vi "RDV-GUI-Compare_Permittivity_calc.vi"() -> ()   [LabVIEW 2020]
doc: "Main viewer, run by hand: loads measurement folders and reference files and compares reflection, impedance and permittivity of every calculation method on graphs and Smith plots, with error analysis. The user picks the folders, the files to compare and the plots to show."
uses:
  RDV-INFO_DATA.ctl
  RDV-UPDATE_IGNORE_LIST.ctl
  Computation/RDC-perm_calc_type.ctl
  RDV-Reflection_Data_viewer.lvclass
  RDV-PRELAUNCH_DATA.ctl
  RDV-XY_GRAPH_REFS.ctl
  RDV-GUI_REFS.ctl
  RDV-PLOT_SETTINGS.ctl
  dedf462c-48f1-4407-ad15-524a3be17598.vi
  Computation/RDC-Reflection_Data_Computation.lvlib
panel:
  out "Selector":T1(graph)
  in  "filter":bool
  in  "unfilter":bool
  in  "Lower Cut-Off":dbl=30000.0 format="%#_13g"
  in  "Calc % error":bool
  in  "Autoscale":bool
  in  "Toggle Plot":bool
  in  "Stop":bool
  in  "Tab Control":T2(tab)
  out "Reflection imag":T1(graph)
  out "Reflection Real":T1(graph)
  out "Impedance imag":T1(graph)
  out "Impedance Real":T1(graph)
  out "Impedance":picture
  out "Permittivity imag":T1(graph)
  out "Permittivity Real":T1(graph)
  out "real error tot":dbl[](array[numeric])
  in  "Reference":u16(ring)=2 items=["00-open0-r", "01-short1-r", "02-water2-r", "03-adblue3-r", "04-eth-124-r", "05-eth-245-r", "06-saline6-r", "07-eth-337-r", "08-eth-488-r", "09-eth-669-r", "10-eth-9610-r", "11-gaba-0111-r", "12-gaba-0512-r", "13-gaba-113-r", "14-iso-1214-r", "15-iso-2515-r", "16-iso-5016-r", "17-iso-9917-r", "18-saline-0p918-r", "19-saline-1-319-r"]
  out "Analyse real":cluster{"Frequency":dbl[], "Perm":dbl[]}[](graph)
  out "Analyse imag":cluster{"Frequency":dbl[], "Perm 2":dbl[]}[](graph)
  out "imag Error":dbl[](array[numeric]) format="%#_6p"
  out "real error":dbl[](array[numeric]) format="%#_6p"
  out "imag error tot":dbl[](array[numeric])
  in  "Data Sets":u16(ring)=1 items=["0-P1_eth-12", "1-P1_eth-24", "2-P1_eth-33", "3-P1_eth-48-2", "4-P1_eth-66", "5-P1_eth-96"]
  in  "Compare Array 2":cluster{"ref":i32, "Set":i32}[](array[cluster])=[{"ref"=0, "Set"=0}, {"ref"=3, "Set"=1}, {"ref"=3, "Set"=2}]
  out "Calculation type":T3[](array[typedef])
  in  "Association set":cluster{"ref":i32, "Set":i32}[](array[cluster])=[{"ref"=3, "Set"=0}, {"ref"=4, "Set"=8}, {"ref"=5, "Set"=10}, {"ref"=7, "Set"=7}, {"ref"=8, "Set"=4}, {"ref"=9, "Set"=3}, {"ref"=10, "Set"=2}, {"ref"=11, "Set"=5}, {"ref"=12, "Set"=6}, {"ref"=13, "Set"=1}, {"ref"=14, "Set"=9}]
  out "compare":T4
  out "Sets of data":string[](array[string])
  out "Total Error real":dbl[](array[numeric])
  out "Total Error Imag":dbl[](array[numeric])
  out "Total Error":dbl[](array[numeric])
  out "All Error imag":dbl[][](array[numeric])
  out "All Error real":dbl[][](array[numeric])
  out "Measurement Param":T5[](array[typedef]) {"lenght" format="%#_6p"; "cap" format="%#_6p"; "Tau" format="%#_6p"}
  in  "Refresh data":bool
  in  "reference paths - Ideal data":path
  in  "common name to remove":string
  in  "max Size":i32=25
  in  "Files for analyses - Data to compare":path
  out "error out":errorcluster
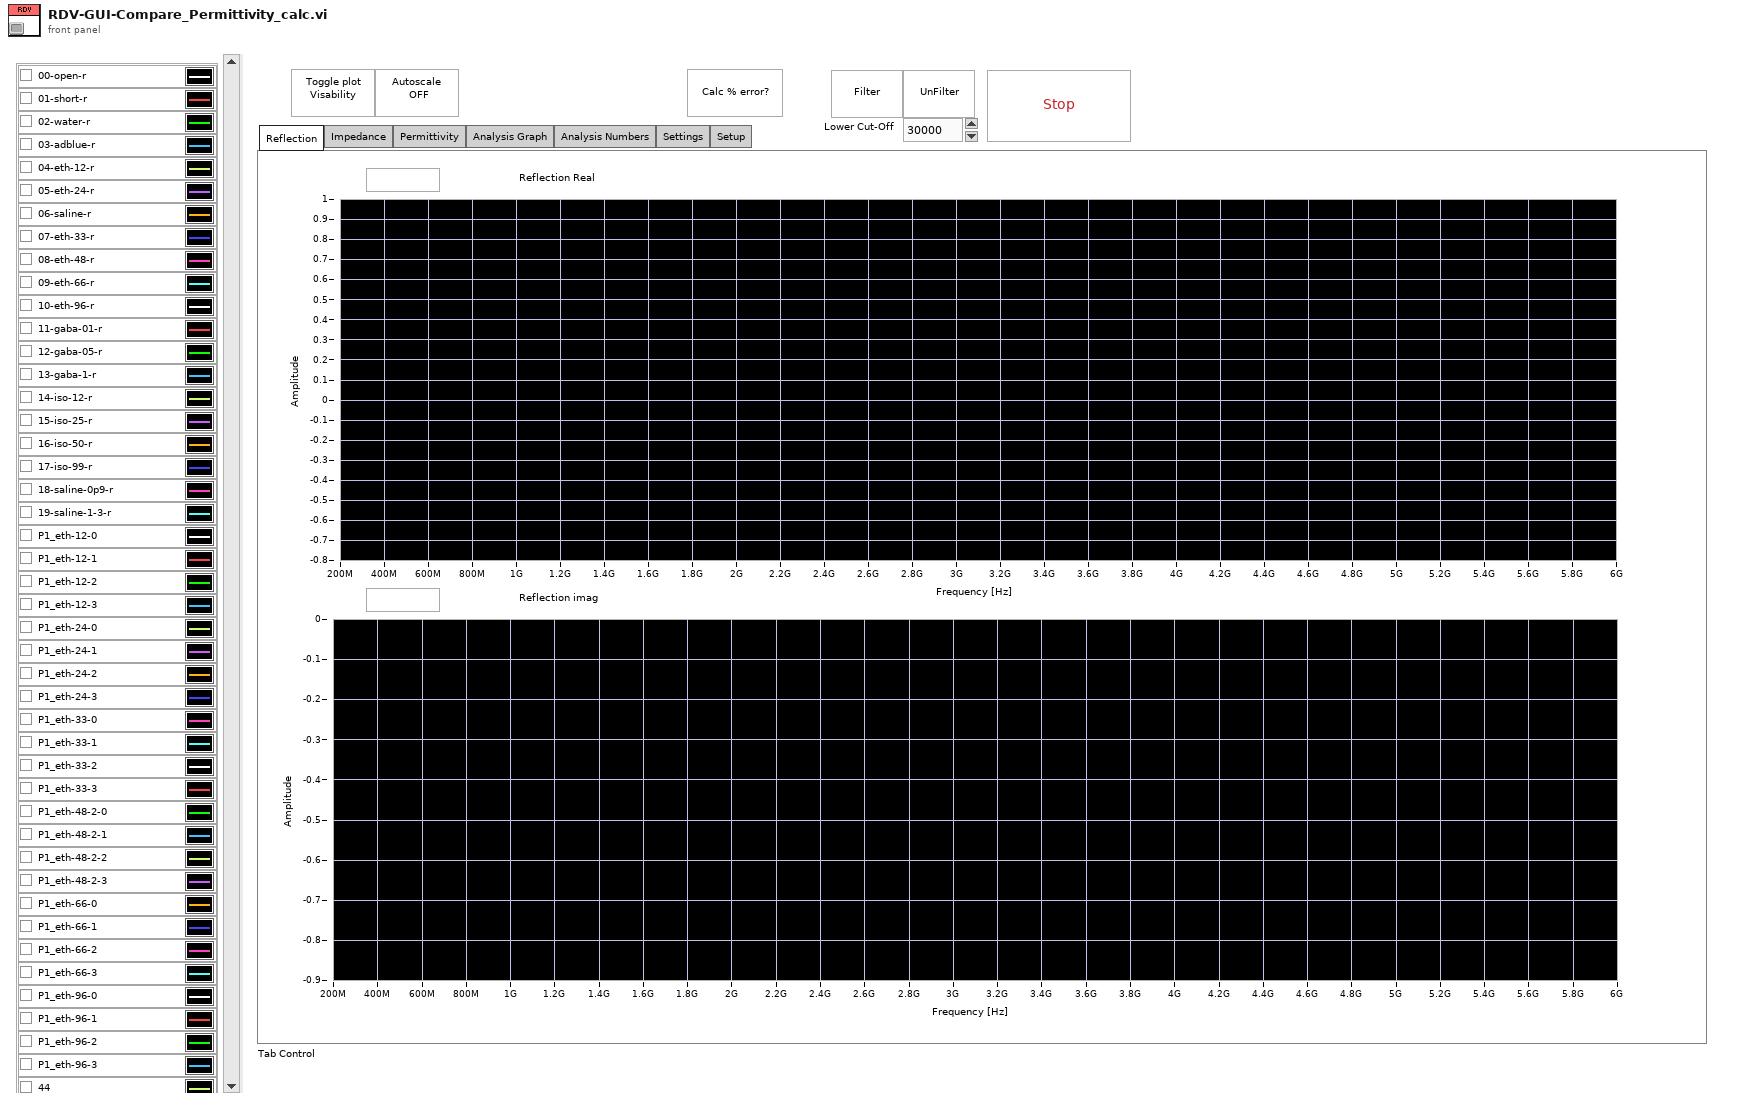
[diagram p1: front panel]
types:
  T1 = cluster{"Frequency":dbl[], "Reflection'":dbl[]}[]
  T2 = enum32{"Reflection", "Impedance", "Permittivity", "Analysis Graph", "Analysis Numbers", "Settings", "Setup"}
  T3 = typedef "RDC-Reflection_Data_Computation.lvlib/RDC-perm_calc_type.ctl" = enum16{"Basic", "Capacative", "Advance", "Bilinear", "Size"}
  T4 = typedef "RDV-Reflection_Data_viewer.lvclass/RDV-UPDATE_IGNORE_LIST.ctl" = string[]
  T5 = typedef "RDV-Reflection_Data_viewer.lvclass/RDV-INFO_DATA.ctl" = cluster{"Name":string, "Tau":dbl, "cap":dbl, "lenght":dbl}
  T6 = typedef "RDV-Reflection_Data_viewer.lvclass/RDV-PLOT_SETTINGS.ctl" = cluster{"common name to remove":string, "Max Size":i32}
  T7 = typedef "RDV-Reflection_Data_viewer.lvclass/RDV-PRELAUNCH_DATA.ctl" = cluster{"XY graph refs":T8, "GUI Refs":T9}
  T8 = typedef "RDV-Reflection_Data_viewer.lvclass/RDV-XY_GRAPH_REFS.ctl" = cluster{"Reflection Real":refnum<vi>, "Reflection Imag":refnum<vi>, "Permittivity Real":refnum<vi>, "Permittivity Imag":refnum<vi>, "Impedance Real":refnum<vi>, "Impedance Imag":refnum<vi>}
  T9 = typedef "RDV-Reflection_Data_viewer.lvclass/RDV-GUI_REFS.ctl" = cluster{"Autoscale":refnum<vi>, "sgl plot Selector":refnum<vi>[], "Smith Plot":refnum<vi>, "plot vis master ":refnum<vi>}
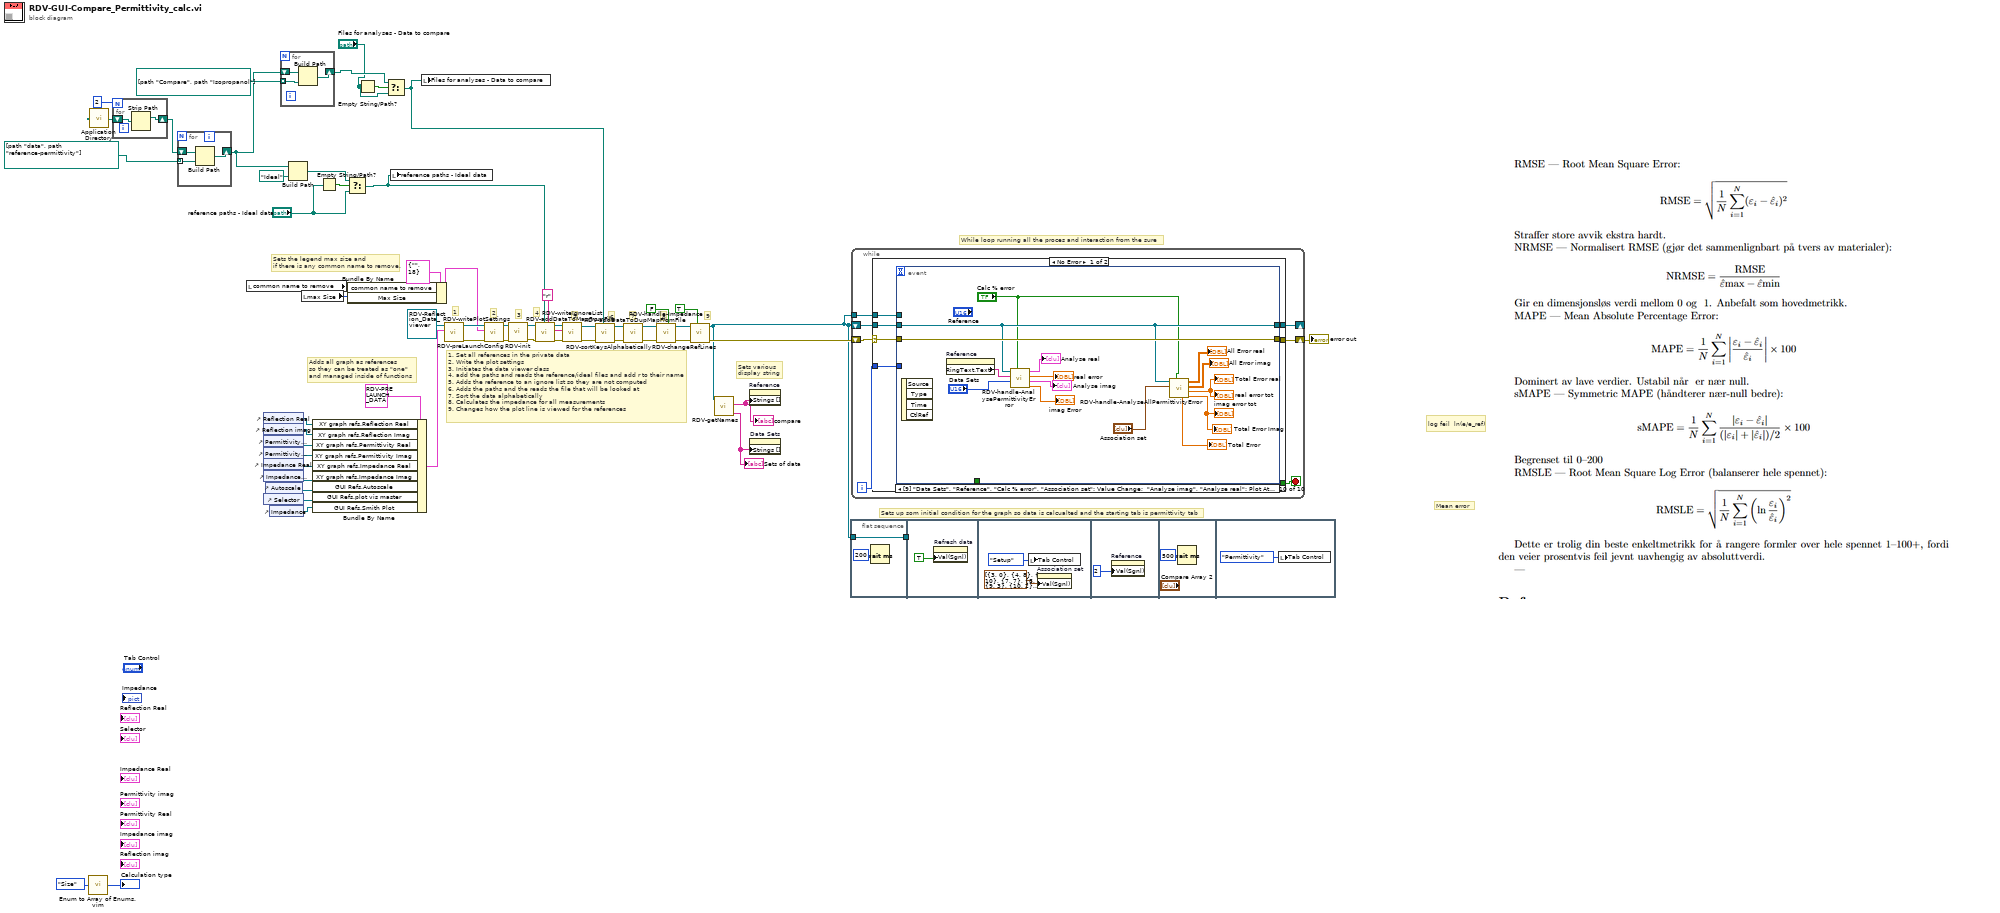
[diagram p0: block diagram]
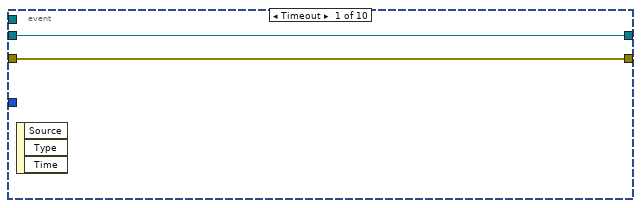
[diagram p2: hidden frame]
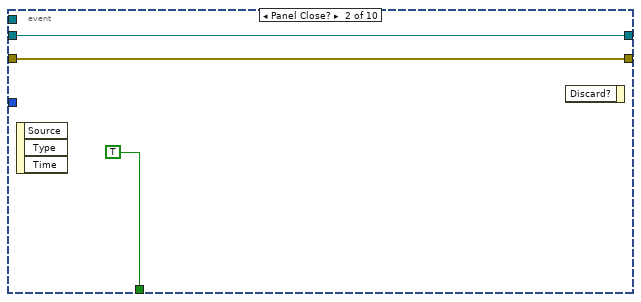
[diagram p3: hidden frame]
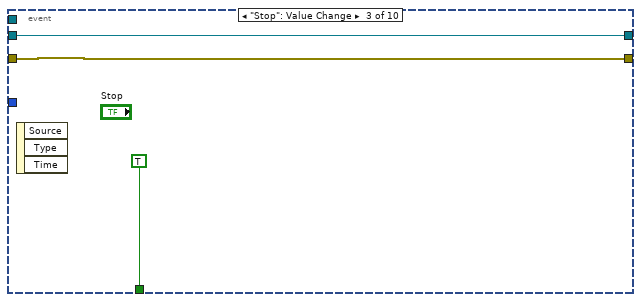
[diagram p4: hidden frame]
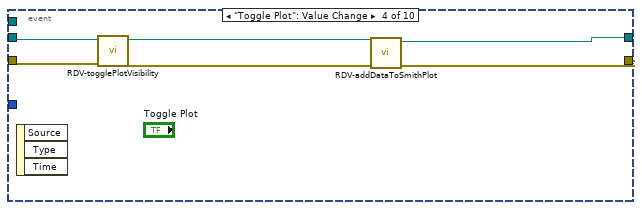
[diagram p5: hidden frame]
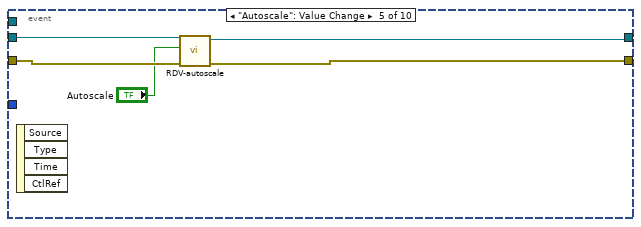
[diagram p6: hidden frame]
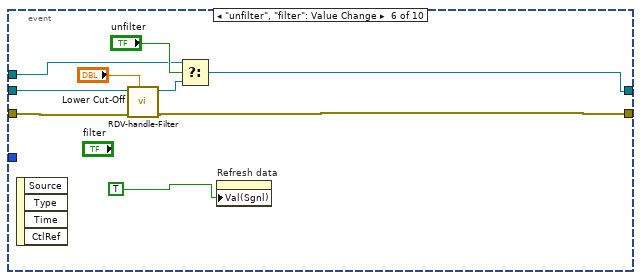
[diagram p7: hidden frame]
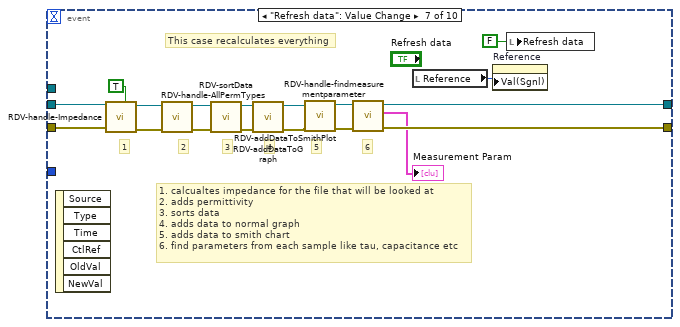
[diagram p8: hidden frame]
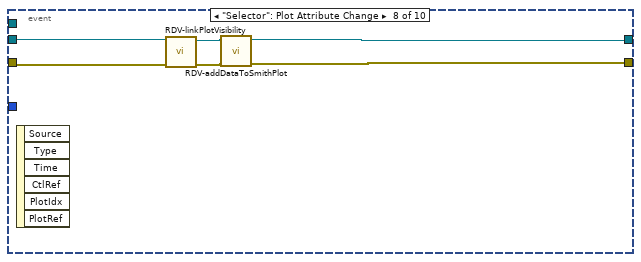
[diagram p9: hidden frame]
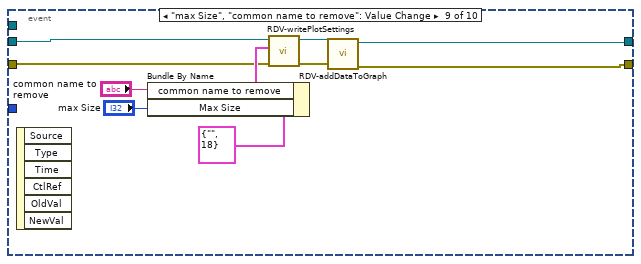
[diagram p10: hidden frame]
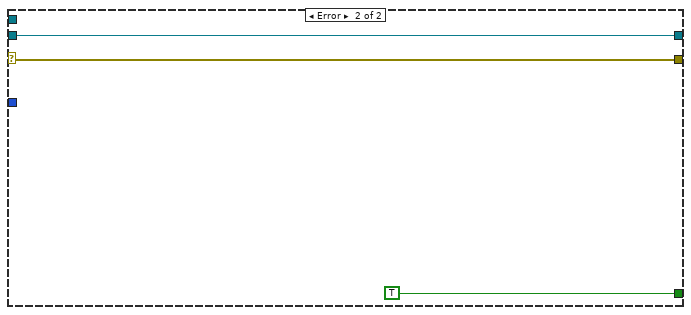
[diagram p11: hidden frame]
diagram:
  # "1. Set all references in the private data\n2. Write the plot settings\n3. Initiates the data viewer class\n4. add the paths and reads the reference/ideal files and add r to their name\n5. Adds the reference to an ignore list so they are not computed\n6. Adds the paths and the reads the file that will be looked at\n7. Sort the data alphabetically\n8. Calculates the impedance for all measurements\n9. Changes how the plot line is viewed for the references"
  # "9"
  # "8"
  # "7"
  # "6"
  # "5"
  # "4"
  # "3"
  # "2"
  # "1"
  # "Sets the legend max size and\nif there is any common name to remove."
  # "Adds all graph as references\nso they can be treated as \"one\"\nand managed inside of functions"
  # "Sets various\ndisplay string"
  # "While loop running all the proces and interaction from the sure"
  # "Sets up som initial condition for the graph so data is calcualted and the starting tab is permittivity tab"
  # "Mean error"
  # "log feil  ln(e/e_ref)"
  n1 = call "Enum to Array of Enums.vim"("enum"=RDC-perm_calc_type."Size" ("Perm calc type")) -> ("array of enums"=→"Calculation type":T3[])
  n2 = call <vilib>:"Application Directory.vi"() -> ("Application Directory"=w13:path)
  n3 = for {
    N: 2 -> [_]
    shift-right: [w60] -> w12
    shift-left: w13 -> [w61]
    n4 = Strip Path(path=w61) -> (stripped path=w60:path)  [unwired: 1 out]
  }
  n5 = for {
    shift-right: [w63] -> w8
    shift-left: w12 -> [w64]
    tunnel: path[] [path "data", path "reference-permittivity"] ("Application Directory") -> [w62] mode=indexing
    n6 = Build Path(base path=w64, name or relative path=w62) -> (appended path=w63:path)
  }
  n7 = local read "common name to remove"() -> (w38:string)
  n8 = control-ref of="Reflection Real"() -> (w52:refnum<vi>)
  n9 = control-ref of="Reflection imag"() -> (w49:refnum<vi>)
  n10 = control-ref of="Permittivity Real"() -> (w48:refnum<vi>)
  n11 = control-ref of="Permittivity imag"() -> (w47:refnum<vi>)
  n12 = control-ref of="Impedance Real"() -> (w46:refnum<vi>)
  n13 = control-ref of="Impedance imag"() -> (w45:refnum<vi>)
  n14 = control-ref of="Selector"() -> (w53:refnum<vi>)
  n15 = control-ref of="Autoscale"() -> (w54:refnum<vi>)
  n16 = control-ref of="Impedance"() -> (w55:refnum<vi>)
  n17 = for {
    shift-right: [w66] -> w4
    shift-left: w8 -> [w67]
    tunnel: path[] [path "Compare", path "Isopropanol"] ("Application Directory") -> [w65] mode=indexing
    n18 = Build Path(base path=w67, name or relative path=w65) -> (appended path=w66:path)
  }
  n19 = Build Path(base path=w8, name or relative path=path "Ideal") -> (appended path=w6:path)
  n20 = local read "max Size"() -> (w37:i32)
  n21 = Bundle By Name(cluster=T7 {"XY graph refs"={"Reflection Real"=refnum, "Reflection Imag"=refnum, "Permittivity Real"=refnum, "Permittivity Imag"=refnum, "Impedance Real"=refnum, "Impedance Imag"=refnum}, "GUI Refs"={"Autoscale"=refnum, "sgl plot Selector"=[], "Smith Plot"=refnum, "plot vis master "=refnum}} ("preLaunch Config"), "XY graph refs.Reflection Real"=w52, "XY graph refs.Reflection Imag"=w49, "XY graph refs.Permittivity Real"=w48, "XY graph refs.Permittivity Imag"=w47, "XY graph refs.Impedance Real"=w46, "XY graph refs.Impedance Imag"=w45, "GUI Refs.Autoscale"=w54, "GUI Refs.plot vis master"=w53, "GUI Refs.Smith Plot"=w55) -> (w56:T7)
  n22 = Empty String/Path?(string/path="reference paths - Ideal data") -> (empty?=w15:bool)
  n23 = Bundle By Name(cluster=T6 {"common name to remove"="", "Max Size"=18} ("Plot Settings"), "common name to remove"=w38, "Max Size"=w37) -> (w39:T6)
  n24 = Select(t=w6, s=w15, f="reference paths - Ideal data") -> (s? t:f=w1:path)
  n25 = Empty String/Path?(string/path="Files for analyses - Data to compare") -> (empty?=w5:bool)
  n26 = Select(t=w4, s=w5, f="Files for analyses - Data to compare") -> (s? t:f=w2:path)
  n27 = local write "reference paths - Ideal data"(w1) -> ()
  n28 = local write "Files for analyses - Data to compare"(w2) -> ()
  n29 = call "RDV-preLaunchConfig.vi"("preLaunch Config"=w56, "RDV-Reflection_Data_viewer in"=refnum<class "RDV-Reflection_Data_viewer.lvclass"> refnum) -> ("error out"=w43:errorcluster, "RDV-Reflection_Data_viewer out"=w44:refnum<class "RDV-Reflection_Data_viewer.lvclass">)  [unwired: 8 in]
  n30 = call "RDV-writePlotSettings.vi"("error in (no error)"=w43, "Plot Settings"=w39, "RDV-Reflection_Data_viewer in"=w44) -> ("error out"=w41:errorcluster, "RDV-Reflection_Data_viewer out"=w42:refnum<class "RDV-Reflection_Data_viewer.lvclass">)  [unwired: 7 in]
  n31 = call "RDV-init.vi"("error in (no error)"=w41, "RDV-Reflection_Data_viewer in"=w42) -> ("error out"=w50:errorcluster, "RDV-Reflection_Data_viewer out"=w51:refnum<class "RDV-Reflection_Data_viewer.lvclass">)  [unwired: 8 in]
  n32 = call "RDV-addDataToMapFromFile.vi"("Add mod"="r", "Folder Path"=w1, "error in (no error)"=w50, "RDV-Reflection_Data_viewer in"=w51) -> ("error out"=w35:errorcluster, "Keys"=w28:string[], "RDV-Reflection_Data_viewer out"=w36:refnum<class "RDV-Reflection_Data_viewer.lvclass">)  [unwired: 5 in]
  n33 = call "RDV-writeIgnoreList.vi"("error in (no error)"=w35, "Keys to ignore"=w28, "RDV-Reflection_Data_viewer in"=w36) -> ("error out"=w32:errorcluster, "RDV-Reflection_Data_viewer out"=w33:refnum<class "RDV-Reflection_Data_viewer.lvclass">)  [unwired: 7 in]
  n34 = call "RDV-addDataToDupMapFromFile.vi"("Folder Path"=w2, "error in (no error)"=w32, "RDV-Reflection_Data_viewer in"=w33) -> ("error out"=w31:errorcluster, "RDV-Reflection_Data_viewer out"=w30:refnum<class "RDV-Reflection_Data_viewer.lvclass">)  [unwired: 6 in, 1 out]
  n35 = call "RDV-sortKeysAlphabetically.vi"("error in (no error)"=w31, "RDV-Reflection_Data_viewer in"=w30) -> ("error out"=w24:errorcluster, "RDV-Reflection_Data_viewer out"=w25:refnum<class "RDV-Reflection_Data_viewer.lvclass">)  [unwired: 7 in, 1 out]
  n36 = call "RDV-handle-Impedance.vi"("Use ignore list (false)"=FALSE, "error in (no error)"=w24, "RDV-Reflection_Data_viewer in"=w25) -> ("error out"=w26:errorcluster, "RDV-Reflection_Data_viewer out"=w27:refnum<class "RDV-Reflection_Data_viewer.lvclass">)  [unwired: 7 in]
  n37 = call "RDV-changeRefLines.vi"("Add lines for ref"=TRUE, "error in (no error)"=w26, "RDV-Reflection_Data_viewer in"=w27) -> ("error out"=w21:errorcluster, "RDV-Reflection_Data_viewer out"=w16:refnum<class "RDV-Reflection_Data_viewer.lvclass">)  [unwired: 7 in]
  n38 = call "RDV-getNames.vi"("RDV-Reflection_Data_viewer in"=w16) -> ("Sets of data"=w18:string[], "Ignore Names"=w22:string[])  [unwired: 8 in, 1 out]
  "compare" <- w22
  "Sets of data" <- w18
  n39 = property on="Reference" class="Ring (strict)"("Strings []"=w22) -> ()  [unwired: 2 in, 2 out]
  n40 = property on="Data Sets" class="Ring (strict)"("Strings []"=w18) -> ()  [unwired: 2 in, 2 out]
  n41 = flat-sequence {
    tunnel: w16 -> [w69]
    tunnel: [w69] -> w59
    tunnel: w59 -> [_]
    frame #0 {
      n42 = Wait (ms)(milliseconds to wait=u32 200) -> ()  [unwired: 1 out]
    }
    frame #1 {
      n43 = property on="Refresh data" class="Bool (strict)"("Val(Sgnl)"=TRUE) -> ()  [unwired: 2 in, 2 out]
    }
    frame #2 {
      n44 = local write "Tab Control"(T2."Setup" ("Tab Control")) -> ()
      n45 = property on="Association set" class="Arr (strict)"("Val(Sgnl)"=cluster{"ref":i32, "Set":i32}[] [{"ref"=3, "Set"=0}, {"ref"=4, "Set"=8}, {"ref"=5, "Set"=10}, {"ref"=7, "Set"=7}, {"ref"=8, "Set"=4}, {"ref"=9, "Set"=3}, {"ref"=10, "Set"=2}, {"ref"=11, "Set"=5}, {"ref"=12, "Set"=6}, {"ref"=13, "Set"=1}, {"ref"=14, "Set"=9}] ("Compare Array")) -> ()  [unwired: 2 in, 2 out]
    }
    frame #3 {
      n46 = property on="Reference" class="Ring (strict)"("Val(Sgnl)"=u16 2 ("Value (Signaling)")) -> ()  [unwired: 2 in, 2 out]
    }
    frame #4 {
      n47 = Wait (ms)(milliseconds to wait=u32 500) -> ()  [unwired: 1 out]
    }
    frame #5 {
      n48 = local write "Tab Control"(T2."Permittivity" ("Tab Control")) -> ()
    }
  }
  n49 = while {
    shift-right: [w81] -> _
    shift-left: w16 -> [w82]
    shift-right: [w79] -> w17
    shift-left: w21 -> [w80]
    tunnel: w16 -> [w76]
    i -> [w77]
    stop <- w78 stop-if-true
    n50 = case shown="No Error" w80 {
      selector: w80 -> [w86 w168]
      tunnel: w82 -> [w87 w169]
      tunnel: [w89 w169] -> w81
      tunnel: [w88 w168] -> w79
      tunnel: [w85 TRUE ("stop")] -> w78
      tunnel: w77 -> [w84 _]
      tunnel: w76 -> [w83 _]
      frame No Error {
        n51 = event shown="[9] \"Data Sets\", \"Reference\", \"Calc % error\", \"Association set\": Value Change;  \"Analyse imag\", \"Analyse real\": Plot Attribute Change" {
          selector: _ -> [_ _ _ _ _ _ _ _ _ _]
          dyn-events: _ -> [_ _ _ _ _ _ _ _ _ _]
          timeout: _ -> [_ _ _ _ _ _ _ _ _ _]
          tunnel: [w91 w93 w96 w98 w105 w111 w120 w136 w143 w153] -> w89
          tunnel: w87 -> [w91 w93 w96 w102 w107 w117 w133 w141 w151 w153]
          tunnel: [w90 w92 w95 w99 w106 w114 w119 w137 w142 w166] -> w88
          tunnel: w86 -> [w90 w92 w95 w103 w108 w115 w132 w140 w146 w166]
          tunnel: [_ TRUE ("Discard?") TRUE ("Discard?") _ _ _ _ _ _ _] -> w85
          tunnel: w84 -> [_ _ _ _ _ _ _ _ _ _]
          tunnel: w83 -> [_ _ _ _ _ w109 _ _ _ _]
          event Timeout {
            n52 = event-data() -> ()  [unwired: 1 in, 3 out]
          }
          event Panel Close? {
            n53 = event-data() -> ()  [unwired: 1 in, 3 out]
            n54 = event-data() -> ()  [unwired: 2 in, 1 out]
          }
          event "Stop": Value Change {
            n55 = event-data() -> ()  [unwired: 1 in, 3 out]
          }
          event "Toggle Plot": Value Change {
            n56 = event-data() -> ()  [unwired: 1 in, 3 out]
            n57 = call "RDV-togglePlotVisibility.vi"("error in (no error)"=w103, "RDV-Reflection_Data_viewer in"=w102) -> ("error out"=w100:errorcluster, "RDV-Reflection_Data_viewer out"=w101:refnum<class "RDV-Reflection_Data_viewer.lvclass">)  [unwired: 8 in]
            n58 = call "RDV-addDataToSmithPlot.vi"("error in (no error)"=w100, "RDV-Reflection_Data_viewer in"=w101) -> ("error out"=w99:errorcluster, "RDV-Reflection_Data_viewer out"=w98:refnum<class "RDV-Reflection_Data_viewer.lvclass">)  [unwired: 8 in]
          }
          event "Autoscale": Value Change {
            n59 = event-data() -> ()  [unwired: 1 in, 4 out]
            n60 = call "RDV-autoscale.vi"("error in (no error)"=w108, "Autoscale"="Autoscale", "RDV-Reflection_Data_viewer in"=w107) -> ("error out"=w106:errorcluster, "RDV-Reflection_Data_viewer out"=w105:refnum<class "RDV-Reflection_Data_viewer.lvclass">)  [unwired: 7 in]
          }
          event "unfilter", "filter": Value Change {
            n61 = event-data() -> ()  [unwired: 1 in, 4 out]
            n62 = call "RDV-handle-Filter.vi"("Lower Cut-Off"="Lower Cut-Off", "error in (no error)"=w115, "RDV-Reflection_Data_viewer in"=w117) -> ("error out"=w114:errorcluster, "RDV-Reflection_Data_viewer out"=w112:refnum<class "RDV-Reflection_Data_viewer.lvclass">)  [unwired: 7 in]
            n63 = Select(t=w109, s="unfilter", f=w112) -> (s? t:f=w111:refnum<class "RDV-Reflection_Data_viewer.lvclass">)
            n64 = property on="Refresh data" class="Bool (strict)"("Val(Sgnl)"=TRUE) -> ()  [unwired: 2 in, 2 out]
          }
          event "Refresh data": Value Change {
            # "6"
            # "This case recalculates everything"
            # "1. calcualtes impedance for the file that will be looked at\n2. adds permittivity\n3. sorts data\n4. adds data to normal graph\n5. adds data to smith chart\n6. find parameters from each sample like tau, capacitance etc"
            # "5"
            # "4"
            # "3"
            # "2"
            # "1"
            n65 = event-data() -> ()  [unwired: 1 in, 6 out]
            n66 = call "RDV-handle-Impedance.vi"("Use ignore list (false)"=TRUE, "error in (no error)"=w132, "RDV-Reflection_Data_viewer in"=w133) -> ("error out"=w130:errorcluster, "RDV-Reflection_Data_viewer out"=w131:refnum<class "RDV-Reflection_Data_viewer.lvclass">)  [unwired: 7 in]
            n67 = call "RDV-handle-AllPermTypes.vi"("error in (no error)"=w130, "RDV-Reflection_Data_viewer in"=w131) -> ("error out"=w128:errorcluster, "RDV-Reflection_Data_viewer out"=w129:refnum<class "RDV-Reflection_Data_viewer.lvclass">)  [unwired: 8 in]
            n68 = call "RDV-sortData.vi"("error in (no error)"=w128, "RDV-Reflection_Data_viewer in"=w129) -> ("error out"=w135:errorcluster, "RDV-Reflection_Data_viewer out"=w127:refnum<class "RDV-Reflection_Data_viewer.lvclass">)  [unwired: 8 in]
            n69 = call "RDV-addDataToGraph.vi"("error in (no error)"=w135, "RDV-Reflection_Data_viewer in"=w127) -> ("error out"=w134:errorcluster, "RDV-Reflection_Data_viewer out"=w126:refnum<class "RDV-Reflection_Data_viewer.lvclass">)  [unwired: 8 in]
            n70 = call "RDV-addDataToSmithPlot.vi"("error in (no error)"=w134, "RDV-Reflection_Data_viewer in"=w126) -> ("error out"=w121:errorcluster, "RDV-Reflection_Data_viewer out"=w122:refnum<class "RDV-Reflection_Data_viewer.lvclass">)  [unwired: 8 in]
            n71 = call "RDV-handle-findmeasurementparameter.vi"("error in (no error)"=w121, "RDV-Reflection_Data_viewer in"=w122) -> ("error out"=w119:errorcluster, "Measurement Parameter"=→"Measurement Param":T5[], "RDV-Reflection_Data_viewer out"=w120:refnum<class "RDV-Reflection_Data_viewer.lvclass">)  [unwired: 7 in]
            n72 = local read "Reference"() -> (w123:u16)
            n73 = property on="Reference" class="Ring (strict)"("Val(Sgnl)"=w123) -> ()  [unwired: 2 in, 2 out]
            n74 = local write "Refresh data"(FALSE ("Refresh data")) -> ()
          }
          event "Selector": Plot Attribute Change {
            n75 = event-data() -> ()  [unwired: 1 in, 6 out]
            n76 = call "RDV-linkPlotVisibility.vi"("error in (no error)"=w140, "RDV-Reflection_Data_viewer in"=w141) -> ("error out"=w138:errorcluster, "RDV-Reflection_Data_viewer out"=w139:refnum<class "RDV-Reflection_Data_viewer.lvclass">)  [unwired: 8 in]
            n77 = call "RDV-addDataToSmithPlot.vi"("error in (no error)"=w138, "RDV-Reflection_Data_viewer in"=w139) -> ("error out"=w137:errorcluster, "RDV-Reflection_Data_viewer out"=w136:refnum<class "RDV-Reflection_Data_viewer.lvclass">)  [unwired: 8 in]
          }
          event "max Size", "common name to remove": Value Change {
            n78 = event-data() -> ()  [unwired: 1 in, 6 out]
            n79 = Bundle By Name(cluster=T6 {"common name to remove"="", "Max Size"=18} ("Plot Settings"), "common name to remove"="common name to remove", "Max Size"="max Size") -> (w149:T6)
            n80 = call "RDV-writePlotSettings.vi"("error in (no error)"=w146, "Plot Settings"=w149, "RDV-Reflection_Data_viewer in"=w151) -> ("error out"=w144:errorcluster, "RDV-Reflection_Data_viewer out"=w145:refnum<class "RDV-Reflection_Data_viewer.lvclass">)  [unwired: 7 in]
            n81 = call "RDV-addDataToGraph.vi"("error in (no error)"=w144, "RDV-Reflection_Data_viewer in"=w145) -> ("error out"=w142:errorcluster, "RDV-Reflection_Data_viewer out"=w143:refnum<class "RDV-Reflection_Data_viewer.lvclass">)  [unwired: 8 in]
          }
          event "Data Sets", "Reference", "Calc % error", "Association set": Value Change; "Analyse imag", "Analyse real": Plot Attribute Change {
            n82 = event-data() -> ()  [unwired: 1 in, 4 out]
            n83 = property on="Reference" class="Ring (strict)"() -> ("RingText.Text"=w165:string)  [unwired: 2 in, 2 out]
            n84 = call "RDV-handle-AnalysePermittivityError.vi"("%?"="Calc % error", "set"="Data Sets", "Reference key"=w165, "RDV-Reflection_Data_viewer in"=w153) -> ("imag Error"=→"imag Error":dbl[], "imag"=→"Analyse imag":cluster{"Frequency":dbl[], "Perm 2":dbl[]}[], "real error"=→"real error":dbl[], "Real"=→"Analyse real":cluster{"Frequency":dbl[], "Perm":dbl[]}[])  [unwired: 4 in]
            n85 = call "RDV-handle-AnalyseAllPermittivityError.vi"("%?"="Calc % error", "Compare Array"="Association set", "RDV-Reflection_Data_viewer in"=w153) -> ("Total Error Imag"=→"imag error tot" →"Total Error Imag":dbl[], "Total Error real"=→"real error tot" →"Total Error real":dbl[], "All Error imag"=→"All Error imag":dbl[][], "All Error real"=→"All Error real":dbl[][], "Total Error"=→"Total Error":dbl[])  [unwired: 4 in]
          }
        }
      }
      frame Error {
      }
    }
  }
  "error out" <- w17
